vi "subXMLGetItemURLFromReferencePath.vi"(9 "Reference path":string, 11 "Root ref":refnum<k20>) -> (1 "Path":path, 2 "Found?":bool, 3 "Refnum out":refnum<k20>)   [LabVIEW 2019, in "SolutionBuilder.lvlib" / "SolutionBuilder.lvclass"]
uses:
  SolutionBuilder.lvclass
  a6dc7d79-757f-4dc2-9727-38c14b9e76cf.vi
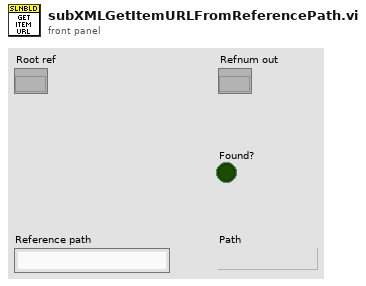
[diagram p1: front panel]
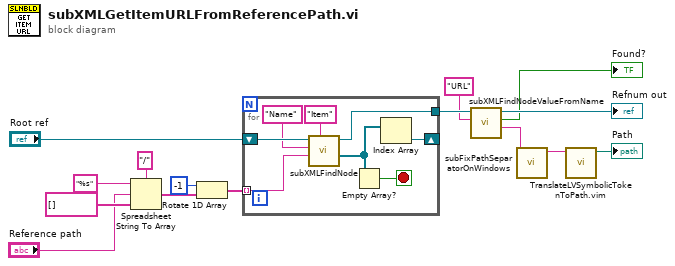
[diagram p0: block diagram]
diagram:
  n1 = Spreadsheet String To Array(delimiter (Tab)="/", format string="%s", spreadsheet string="Reference path", array type (2D Dbl)=string[] [] ("Names")) -> (array=w7:string[])
  n2 = Rotate 1D Array(1:w7, 2:-1 ("n")) -> (0:w5:string[])
  n3 = for {
    shift-right: [w18] -> _
    shift-left: "Root ref" -> [w23]
    tunnel: w5 -> [w22] mode=indexing
    tunnel: [w16] -> w10
    stop <- w17 stop-if-true
    n4 = call "subXMLFindNode.vi"("Node name"="Item", "Property value"=w22, "Property name"="Name", "Refnum in"=w23) -> ("Nodes"=w19:refnum<k20>[], "Refnum"=w16:refnum<k20>)  [unwired: 6 in]
    n5 = Empty Array?(array=w19) -> (empty?=w17:bool)
    n6 = Index Array(array=w19) -> (element=w18:refnum<k20>)  [unwired: 1 in]
  }
  n7 = call "subXMLFindNodeValueFromName.vi"("Property name"="URL", "Refnum in"=w10) -> ("Value"=w3:string, "Found?"=→"Found?":bool, "Refnum out"=→"Refnum out":refnum<k20>)  [unwired: 7 in]
  n8 = call "subFixPathSeparatorOnWindows.vi"("Value"=w3) -> ("fixed path"=w2:string)  [unwired: 10 in]
  n9 = call "TranslateLVSymbolicTokenToPath.vim"("Path in"=w2) -> ("Path"=→"Path":path)  [unwired: 10 in]
